vi "Read current vs temperature_3ch_2.1.vi"(8 "stop":bool) -> (0 "X3":cluster{"Y":dbl[], "Y":dbl[]}[](graph), 1 "Zx 4":cluster{"Y":dbl[], "Y":dbl[]}[](graph), 2 "Zx 3":cluster{"Y":dbl[], "Y":dbl[]}[](graph), 3 "Temp vs Time":cluster{"Y":dbl[], "Y":dbl[]}[](graph), 4 "i X":cluster{"Y":dbl[], "Y":dbl[]}[](graph), 5 "X 2":cluster{"Y":dbl[], "Y":dbl[]}[](graph))   [LabVIEW 2013]
uses:
  PPMS_remote/branches/sim-JL/Simulate.glb.vi
  lockin/branches/PPMS-demomode-JL/Lock-in Globles.vi
  SubVI/ITX_Global.vi
panel:
  in  "Tab Control":T1(tab)
  in  "Lockins":u16[](array[ring]) items=["Lock-in #1", "Lock-in #2", "Lock-in #3", "Lock-in #4"]
  out "OSC Configuration":T2(array[cluster])=[{"Signal Type"=enum."Sine Wave", "DC"=0.0005, "Amplitude"=0.001, "frequency"=1.346, "Phase"=0.0}, {"Signal Type"=enum."Sine Wave", "DC"=0.0, "Amplitude"=0.0, "frequency"=1.346, "Phase"=0.0}, {"Signal Type"=enum."Sine Wave", "DC"=0.0, "Amplitude"=0.0, "frequency"=1.346, "Phase"=0.0}, {"Signal Type"=enum."Sine Wave", "DC"=0.0, "Amplitude"=0.0, "frequency"=1.346, "Phase"=0.0}] {"frequency" format="%0.2p"; "Amplitude" format="%0.2p"; "DC" format="%.2p"}
  in  "milliseconds to wait":u32=1000
  in  "Comments":string="SA02610M 20130128\ncool down\n"
  out "Connected":string="I-:4\nV2+:28\nI+:1\nV1+:2\nV-:3\nV2-:5\n"
  out "i Y":cluster{"Y":dbl[], "Y":dbl[]}[](graph)
  out "i X 3":cluster{"Y":dbl[], "Y":dbl[]}[](graph)
  out "i Y 3":cluster{"Y":dbl[], "Y":dbl[]}[](graph)
  out "Y 2":cluster{"Y":dbl[], "Y":dbl[]}[](graph)
  out "Y3":cluster{"Y":dbl[], "Y":dbl[]}[](graph)
  out "Zy 3":cluster{"Y":dbl[], "Y":dbl[]}[](graph)
  out "Zy 4":cluster{"Y":dbl[], "Y":dbl[]}[](graph)
  out "i X 2":cluster{"Y":dbl[], "Y":dbl[]}[](graph)
  out "i X 4":cluster{"Y":dbl[], "Y":dbl[]}[](graph)
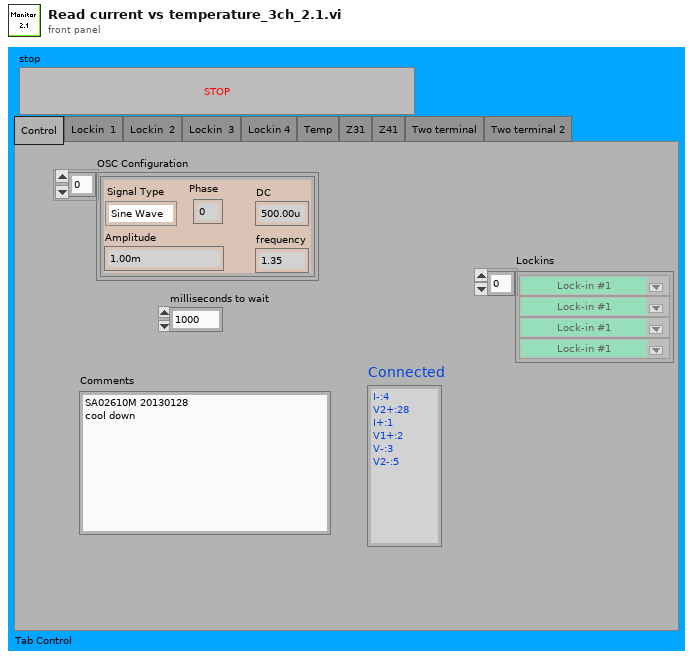
[diagram p1: front panel]
types:
  T1 = enum32{"Control", "Lockin  1", "Lockin  2", "Lockin  3", "Lockin 4", "Temp", "Z31", "Z41", "Two terminal", "Two terminal 2"}
  T2 = cluster{"Signal Type":enum16{"Sine Wave", "Triangle Wave", "Square Wave", "Sawtooth Wave"}, "DC":dbl, "Amplitude":dbl, "frequency":dbl, "Phase":dbl}[]
  T3 = cluster{"Signal Type":enum16{"Sine Wave", "Triangle Wave", "Square Wave", "Sawtooth Wave"}, "DC":dbl, "Amplitude":dbl, "frequency":dbl, "Phase":dbl}
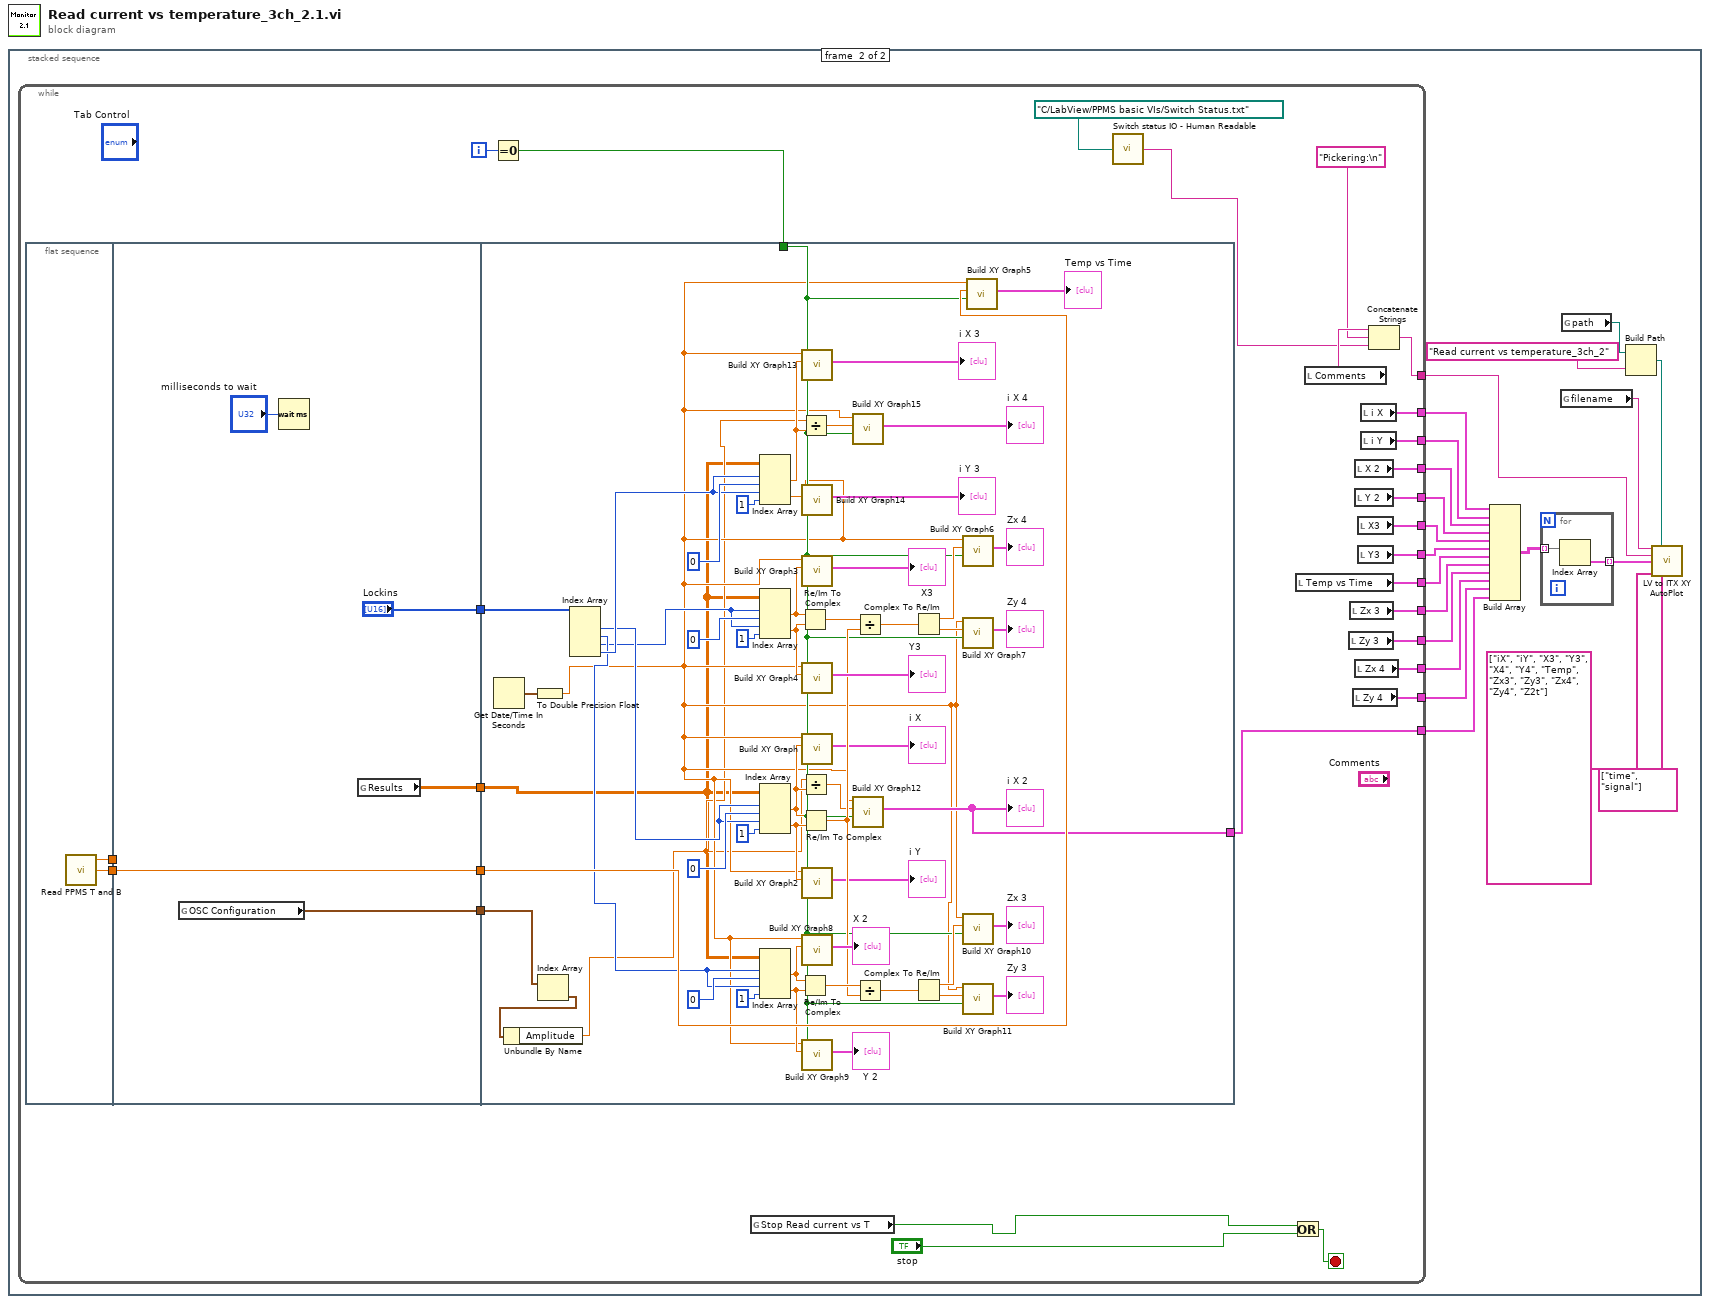
[diagram p0: block diagram]
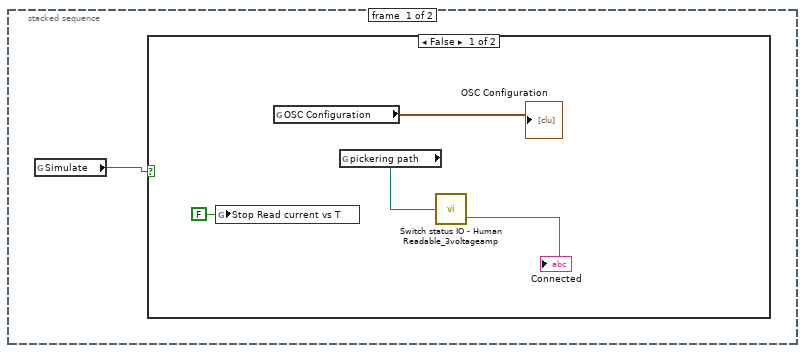
[diagram p2: hidden frame]
diagram:
  n1 = stacked-sequence {
    frame #0 {
      n2 = global read "Simulate.glb.vi" "Simulate"() -> (w1:bool)
      n3 = case shown="False" w1 {
        frame False {
          n4 = global write "Lock-in Globles.vi" "Stop Read current vs T"(FALSE ("Stop Read current vs T")) -> ()
          n5 = global read "Lock-in Globles.vi" "OSC Configuration"() -> (→"OSC Configuration":T2)
          n6 = global read "ITX_Global.vi" "pickering path"() -> (w2:path)
          n7 = call "Switch status IO - Human Readable_3voltageamp.vi"("Switch status"=w2) -> ("String"=→"Connected":string)  [unwired: 3 in]
        }
        frame True {
        }
      }
    }
    frame #1 {
      n8 = while {
        tunnel: [w49] -> w26
        tunnel: [w48] -> w25
        tunnel: [w47] -> w24
        tunnel: [w46] -> w23
        tunnel: [w45] -> w22
        tunnel: [w44] -> w21
        tunnel: [w43] -> w20
        tunnel: [w42] -> w19
        tunnel: [w41] -> w18
        tunnel: [w40] -> w17
        tunnel: [w39] -> w16
        tunnel: [w37] -> w12
        tunnel: [w32] -> w6
        i -> [w54]
        stop <- w51 stop-if-true
        n9 = flat-sequence {
          tunnel: [w58] -> w55
          tunnel: [w57] -> w52
          tunnel: [w62] -> w56
          tunnel: w55 -> [w62]
          tunnel: w52 -> [_]
          tunnel: [w61] -> w31
          tunnel: ["Lockins"] -> w30
          tunnel: [w59] -> w29
          tunnel: w56 -> [w102]
          tunnel: w53 -> [w76]
          tunnel: [w84] -> w32
          tunnel: w31 -> [w68]
          tunnel: w30 -> [w65]
          tunnel: w29 -> [w64]
          frame #0 {
            n10 = call "Read PPMS T and B.vi"() -> ("Temperature"=w58:dbl, "Time"=w57:dbl)  [unwired: 3 in, 1 out]
          }
          frame #1 {
            n11 = global read "Lock-in Globles.vi" "OSC Configuration"() -> (w61:T2)
            n12 = Wait (ms)(milliseconds to wait="milliseconds to wait") -> ()  [unwired: 1 out]
            n13 = global read "Lock-in Globles.vi" "Results"() -> (w59:dbl[][])
          }
          frame #2 {
            n14 = Get Date/Time In Seconds() -> (seconds since 1Jan1904=w70:timestamp)
            n15 = To Double Precision Float(number=w70) -> (double precision float=w69:dbl)
            n16 = Index Array(array=w68) -> (element=w67:T3)  [unwired: 1 in]
            n17 = Unbundle By Name(w67) -> ("Amplitude"=w66:dbl)
            n18 = Index Array(array=w65) -> (element #1=w73:u16, element #2=w72:u16, element #3=w71:u16, element #4=w74:u16)  [unwired: 4 in]
            n19 = Index Array(array=w64, index (row) #1=w74, index (col) #1=0 ("disabled index (col)"), index (row) #2=w74, index (col) #2=1 ("disabled index (col)")) -> (element #1=w78:dbl, element #2=w79:dbl)
            n20 = Index Array(array=w64, index (row) #1=w71, index (col) #1=0 ("disabled index (col)"), index (row) #2=w71, index (col) #2=1 ("disabled index (col)")) -> (element #1=w110:dbl, element #2=w109:dbl)
            n21 = Index Array(array=w64, index (row) #1=w73, index (col) #1=0 ("disabled index (col)"), index (row) #2=w73, index (col) #2=1 ("disabled index (col)")) -> (element #1=w86:dbl, element #2=w111:dbl)
            n22 = Index Array(array=w64, index (row) #1=w72, index (col) #1=0 ("disabled index (col)"), index (row) #2=w72, index (col) #2=1 ("disabled index (col)")) -> (element #1=w97:dbl, element #2=w96:dbl)
            n23 = Re/Im To Complex(1:w109, 2:w110) -> (0:w108:cdb)
            n24 = Re/Im To Complex(1:w96, 2:w97) -> (0:w95:cdb)
            n25 = Divide(x=w66, y=w78) -> (x/y=w77:dbl)
            n26 = Divide(x=w66, y=w86) -> (x/y=w85:dbl)
            n27 = Re/Im To Complex(1:w111, 2:w86) -> (0:w94:cdb)
            n28 = call "Build XY Graph13"("Reset"=w76, "Y Input"=w78, "X Input"=w69) -> ("XY Graph"=→"i X 3":cluster{"Y":dbl[], "Y":dbl[]}[])  [unwired: 2 in, 6 out]
            n29 = call "Build XY Graph14"("Reset"=w76, "Y Input"=w79, "X Input"=w69) -> ("XY Graph"=→"i Y 3":cluster{"Y":dbl[], "Y":dbl[]}[])  [unwired: 2 in, 6 out]
            n30 = call "Build XY Graph3"("Reset"=w76, "Y Input"=w110, "X Input"=w69) -> ("XY Graph"=→"X3":cluster{"Y":dbl[], "Y":dbl[]}[])  [unwired: 2 in, 6 out]
            n31 = call "Build XY Graph4"("Reset"=w76, "Y Input"=w109, "X Input"=w69) -> ("XY Graph"=→"Y3":cluster{"Y":dbl[], "Y":dbl[]}[])  [unwired: 2 in, 6 out]
            n32 = call "Build XY Graph"("Reset"=w76, "Y Input"=w86, "X Input"=w69) -> ("XY Graph"=→"i X":cluster{"Y":dbl[], "Y":dbl[]}[])  [unwired: 2 in, 6 out]
            n33 = call "Build XY Graph2"("Reset"=w76, "Y Input"=w111, "X Input"=w69) -> ("XY Graph"=→"i Y":cluster{"Y":dbl[], "Y":dbl[]}[])  [unwired: 2 in, 6 out]
            n34 = call "Build XY Graph8"("Reset"=w76, "Y Input"=w97, "X Input"=w69) -> ("XY Graph"=→"X 2":cluster{"Y":dbl[], "Y":dbl[]}[])  [unwired: 2 in, 6 out]
            n35 = call "Build XY Graph9"("Reset"=w76, "Y Input"=w96, "X Input"=w69) -> ("XY Graph"=→"Y 2":cluster{"Y":dbl[], "Y":dbl[]}[])  [unwired: 2 in, 6 out]
            n36 = call "Build XY Graph15"("Reset"=w76, "Y Input"=w77, "X Input"=w69) -> ("XY Graph"=→"i X 4":cluster{"Y":dbl[], "Y":dbl[]}[])  [unwired: 2 in, 6 out]
            n37 = call "Build XY Graph12"("Reset"=w76, "Y Input"=w85, "X Input"=w69) -> ("XY Graph"=w84:cluster{"Y":dbl[], "Y":dbl[]}[])  [unwired: 2 in, 6 out]
            "i X 2" <- w84
            n38 = Divide(x=w108, y=w94) -> (x/y=w107:cdb)
            n39 = Divide(x=w95, y=w94) -> (x/y=w93:cdb)
            n40 = Complex To Re/Im(x + iy=w107) -> (x=w105:dbl, y=w106:dbl)
            n41 = Complex To Re/Im(x + iy=w93) -> (x=w92:dbl, y=w91:dbl)
            n42 = call "Build XY Graph6"("Reset"=w76, "Y Input"=w105, "X Input"=w69) -> ("XY Graph"=→"Zx 4":cluster{"Y":dbl[], "Y":dbl[]}[])  [unwired: 2 in, 6 out]
            n43 = call "Build XY Graph7"("Reset"=w76, "Y Input"=w106, "X Input"=w69) -> ("XY Graph"=→"Zy 4":cluster{"Y":dbl[], "Y":dbl[]}[])  [unwired: 2 in, 6 out]
            n44 = call "Build XY Graph10"("Reset"=w76, "Y Input"=w92, "X Input"=w69) -> ("XY Graph"=→"Zx 3":cluster{"Y":dbl[], "Y":dbl[]}[])  [unwired: 2 in, 6 out]
            n45 = call "Build XY Graph11"("Reset"=w76, "Y Input"=w91, "X Input"=w69) -> ("XY Graph"=→"Zy 3":cluster{"Y":dbl[], "Y":dbl[]}[])  [unwired: 2 in, 6 out]
            n46 = call "Build XY Graph5"("Reset"=w76, "Y Input"=w102, "X Input"=w69) -> ("XY Graph"=→"Temp vs Time":cluster{"Y":dbl[], "Y":dbl[]}[])  [unwired: 2 in, 6 out]
          }
        }
        n47 = Equal To 0?(x=w54) -> (x = 0?=w53:bool)
        n48 = global read "Lock-in Globles.vi" "Stop Read current vs T"() -> (w33:bool)
        n49 = call "Switch status IO - Human Readable.vi"("Switch status"=path "C:/LabView/PPMS basic VIs/Switch Status.txt") -> ("String"=w34:string)
        n50 = Or(x=w33, y="stop") -> (x .or. y?=w51:bool)
        n51 = local read "Temp vs Time"() -> (w43:cluster{"Y":dbl[], "Y":dbl[]}[])
        n52 = local read "Comments"() -> (w36:string)
        n53 = local read "Zy 3"() -> (w41:cluster{"Y":dbl[], "Y":dbl[]}[])
        n54 = local read "Zx 3"() -> (w42:cluster{"Y":dbl[], "Y":dbl[]}[])
        n55 = local read "Zy 4"() -> (w39:cluster{"Y":dbl[], "Y":dbl[]}[])
        n56 = local read "X 2"() -> (w47:cluster{"Y":dbl[], "Y":dbl[]}[])
        n57 = local read "Y 2"() -> (w46:cluster{"Y":dbl[], "Y":dbl[]}[])
        n58 = local read "Zx 4"() -> (w40:cluster{"Y":dbl[], "Y":dbl[]}[])
        n59 = local read "X3"() -> (w45:cluster{"Y":dbl[], "Y":dbl[]}[])
        n60 = local read "Y3"() -> (w44:cluster{"Y":dbl[], "Y":dbl[]}[])
        n61 = local read "i X"() -> (w49:cluster{"Y":dbl[], "Y":dbl[]}[])
        n62 = local read "i Y"() -> (w48:cluster{"Y":dbl[], "Y":dbl[]}[])
        n63 = Concatenate Strings(w36, "Pickering:\n" ("string"), w34) -> (w37:string)
      }
      n64 = Build Array(w26, w25, w24, w23, w22, w21, w20, w19, w18, w17, w16, w6) -> (w15:cluster{"Y":dbl[], "Y":dbl[]}[][])
      n65 = for {
        tunnel: w15 -> [w28] mode=indexing
        tunnel: [w27] -> w14 mode=indexing
        n66 = Index Array(array=w28) -> (element=w27:cluster{"Y":dbl[], "Y":dbl[]})  [unwired: 1 in]
      }
      n67 = global read "ITX_Global.vi" "filename"() -> (w13:string)
      n68 = global read "ITX_Global.vi" "path"() -> (w9:path)
      n69 = Build Path(base path=w9, name or relative path="Read current vs temperature_3ch_2") -> (appended path=w8:path)
      n70 = call <userlib>:"LV to ITX XY AutoPlot.vi"("filename"=w13, "path"=w8, "Notes"=w12, "XY Array"=w14, "wavenames (.Vx, etc)"=string[] ["iX", "iY", "X3", "Y3", "X4", "Y4", "Temp", "Zx3", "Zy3", "Zx4", "Zy4", "Z2t"], "X,Y Labels"=string[] ["time", "signal"]) -> ()  [unwired: 9 in, 1 out]
    }
  }
